vi "Player_Move.vi"(0 "State":T1={"Tick"=0, "Phase"=0, "PhaseTicks"=0, "Level"=1, "Room"=0, "X10"=0, "Y10"=0, "VY10"=0, "Mode"=0, "Facing"=0, "Run"=0, "Vert"=0, "StandY"=0, "EntryX10"=0, "EntryY10"=0, "EntryMode"=0, "Lives"=4, "Score"=0, "NextLife"=10000, "KeyR"=0, "KeyB"=0, "KeyY"=0, "Torch"=FALSE, "FloorPhase"=0, "Dead"=FALSE, "LevelStart"=FALSE, "Quit"=FALSE, "Sound"=0, "Seed"=12345, "DemoStep"=0, "Tiles"=[], "World"=[], "Enemies"=[], "Highscores"=[], "Name"=[0, 0, 0], "Cursor"=0}, 5 "Jump":bool, 11 "error in":errorcluster) -> (4 "State out":T1={"Tick"=0, "Phase"=0, "PhaseTicks"=0, "Level"=1, "Room"=0, "X10"=0, "Y10"=0, "VY10"=0, "Mode"=0, "Facing"=0, "Run"=0, "Vert"=0, "StandY"=0, "EntryX10"=0, "EntryY10"=0, "EntryMode"=0, "Lives"=4, "Score"=0, "NextLife"=10000, "KeyR"=0, "KeyB"=0, "KeyY"=0, "Torch"=FALSE, "FloorPhase"=0, "Dead"=FALSE, "LevelStart"=FALSE, "Quit"=FALSE, "Sound"=0, "Seed"=12345, "DemoStep"=0, "Tiles"=[], "World"=[], "Enemies"=[], "Highscores"=[], "Name"=[0, 0, 0], "Cursor"=0}, 15 "error out":errorcluster)   [LabVIEW 2020, in "GH_Engine.lvlib"]
doc: "Moves Claude by one tick: the step sideways (walking in Mode 0 and 2, conveyor push in Mode 0, stopped by a wall), then the mode: Move_Ground (0), Move_Ladder (1), Move_Air (2) or Move_Pole (3), all inline. Facing follows Run; StandY = last firm stand (for the fall height). Positions are tenths of a pixel."
uses:
  GH_Engine.lvlib
  Level/GH_Level.lvlib
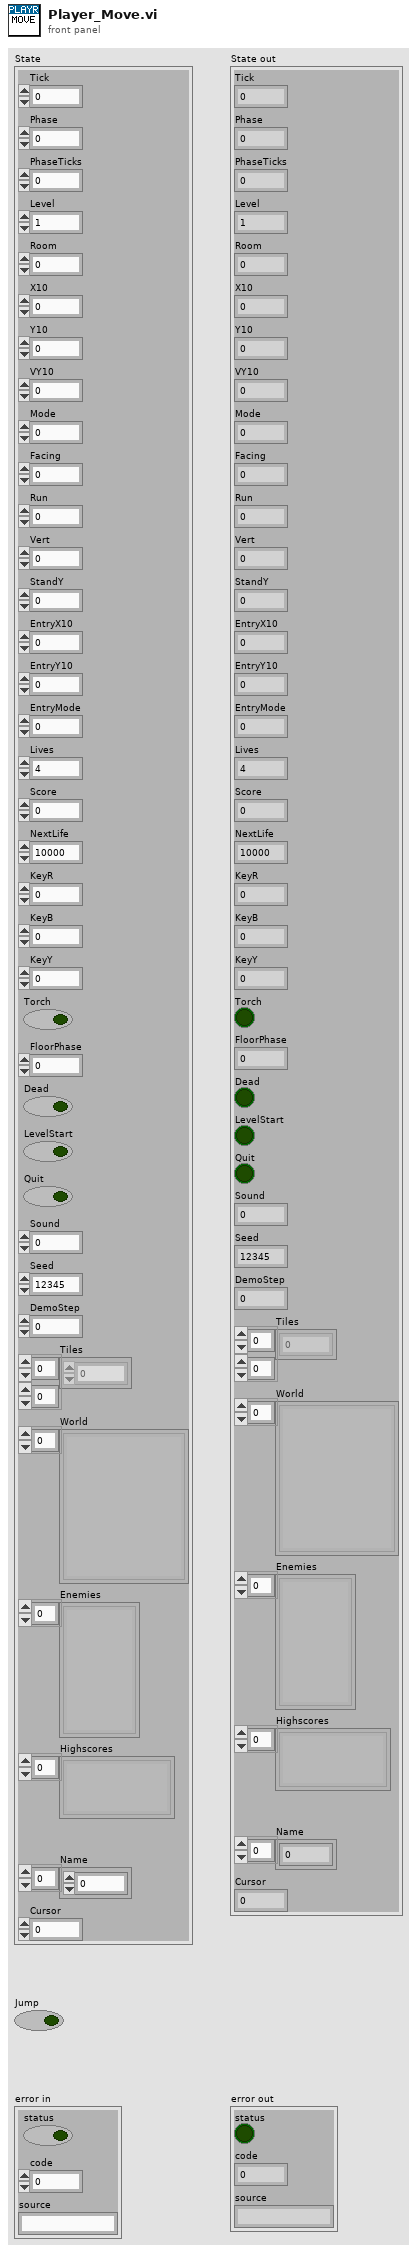
[diagram p1: front panel]
types:
  T1 = cluster{"Tick":u32, "Phase":i32, "PhaseTicks":i32, "Level":i32, "Room":i32, "X10":i32, "Y10":i32, "VY10":i32, "Mode":i32, "Facing":i32, "Run":i32, "Vert":i32, "StandY":i32, "EntryX10":i32, "EntryY10":i32, "EntryMode":i32, "Lives":i32, "Score":i32, "NextLife":i32, "KeyR":i32, "KeyB":i32, "KeyY":i32, "Torch":bool, "FloorPhase":i32, "Dead":bool, "LevelStart":bool, "Quit":bool, "Sound":i32, "Seed":u32, "DemoStep":i32, "Tiles":u8[][], "World":cluster{"ID":string, "Depth":i32, "Column":i32, "Tiles":u8[][]}[], "Enemies":cluster{"Kind":i32, "X10":i32, "Y10":i32, "Dir":i32, "Mode":i32}[], "Highscores":cluster{"Score":i32, "Name":string}[], "Name":i32[], "Cursor":i32}
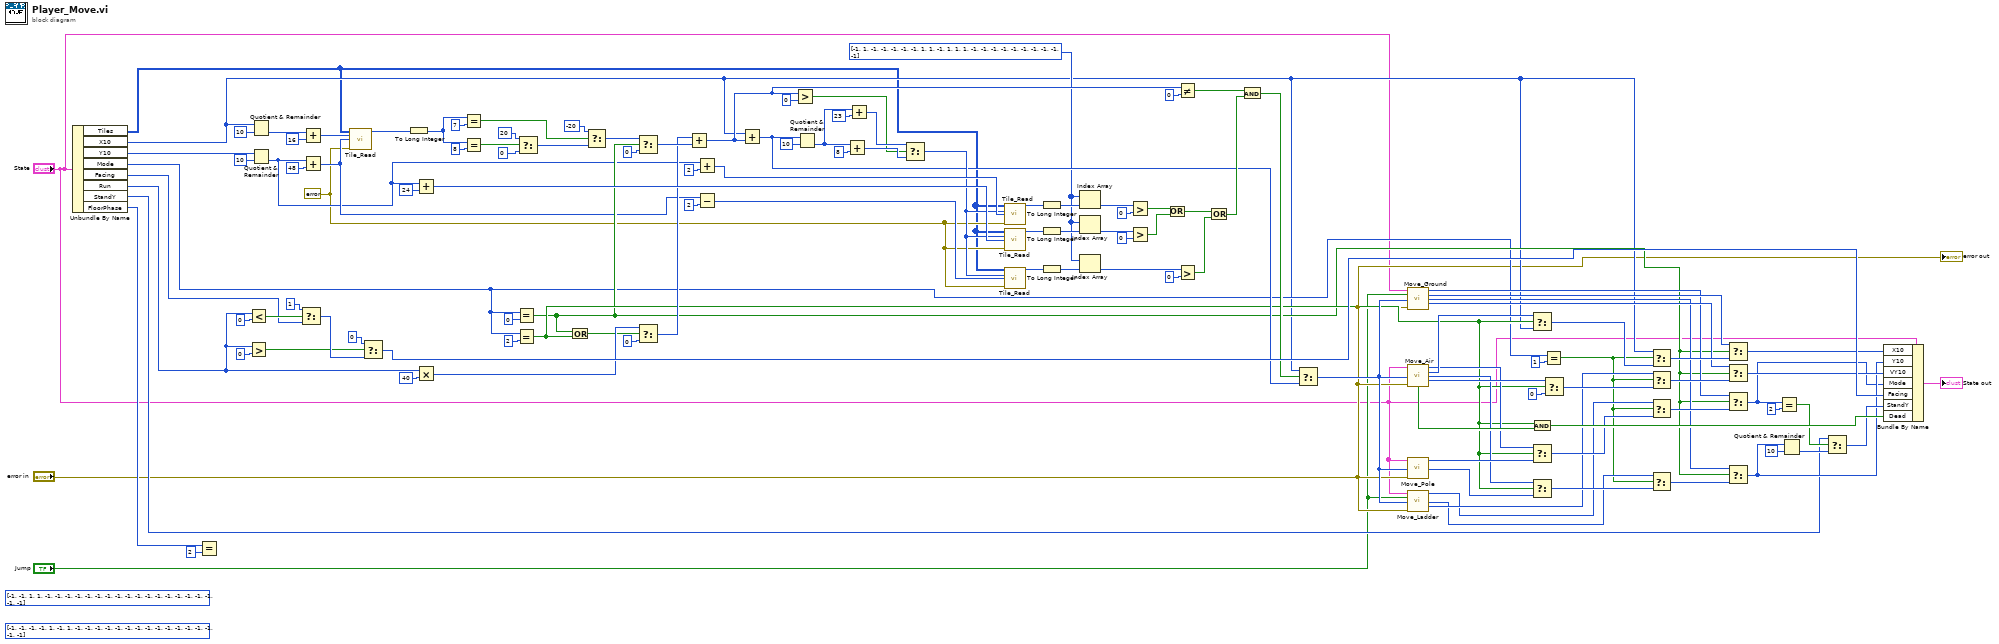
[diagram p0: block diagram]
diagram:
  w14 = errorcluster {"status"=FALSE, "code"=0, "source"=""} ("no error")
  (unwired) i32[] [-1, -1, -1, -1, 1, -1, 1, -1, -1, -1, -1, -1, -1, -1, -1, -1, -1, -1, -1, -1, -1, -1, -1] ("Ladder or rope")
  (unwired) i32[] [-1, -1, 1, 1, -1, -1, -1, -1, -1, -1, -1, -1, -1, -1, -1, -1, -1, -1, -1, -1, -1, -1, -1] ("Thin floor")
  w12 = i32[] [-1, 1, -1, -1, -1, -1, -1, 1, 1, -1, 1, 1, 1, -1, -1, -1, -1, -1, -1, -1, -1, -1, -1] ("Solid")
  n1 = Unbundle By Name("State") -> ("Tiles"=w4:u8[][], "X10"=w5:i32, "Y10"=w6:i32, "Mode"=w7:i32, "Facing"=w8:i32, "Run"=w9:i32, "StandY"=w10:i32, "FloorPhase"=w11:i32)
  n2 = Equal?(x=w11, y=2) -> ()  [unwired: 1 out]
  n3 = Less?(x=w9, y=0) -> (x < y?=w121:bool)
  n4 = Greater?(x=w9, y=0) -> (0:w118:bool)
  n5 = Quotient & Remainder(x=w5, y=10) -> (floor(x/y)=w16:i32)  [unwired: 1 out]
  n6 = Quotient & Remainder(x=w6, y=10) -> (floor(x/y)=w18:i32)  [unwired: 1 out]
  n7 = Select(t=1, s=w121, f=w8) -> (s? t:f=w123:i32)
  n8 = Add(x=w16, y=16) -> (x+y=w28:i32)
  n9 = Add(x=w18, y=48) -> (x+y=w20:i32)
  n10 = call "Tile_Read.vi"("Tiles"=w4, "X"=w28, "Y"=w20, "error in"=w14) -> ("Tile"=w29:u8)  [unwired: 10 in, 1 out]
  n11 = Select(t=0, s=w118, f=w123) -> (s? t:f=w124:i32)
  n12 = To Long Integer(number=w29) -> (32bit integer=w30:i32)
  n13 = Add(x=w18, y=24) -> (x+y=w66:i32)
  n14 = Multiply(x=w9, y=40) -> (x*y=w42:i32)
  n15 = Equal?(x=w30, y=7) -> (x = y?=w32:bool)
  n16 = Equal?(x=w30, y=8) -> (x = y?=w35:bool)
  n17 = Equal?(x=w7, y=0) -> (x = y?=w22:bool)
  n18 = Equal?(x=w7, y=2) -> (x = y?=w26:bool)
  n19 = Select(t=20, s=w35, f=0) -> (s? t:f=w38:i32)
  n20 = Or(x=w22, y=w26) -> (x .or. y?=w40:bool)
  n21 = Select(t=-20, s=w32, f=w38) -> (s? t:f=w39:i32)
  n22 = Select(t=w39, s=w22, f=0) -> (s? t:f=w46:i32)
  n23 = Select(t=w42, s=w40, f=0) -> (s? t:f=w44:i32)
  n24 = Add(x=w44, y=w46) -> (x+y=w47:i32)
  n25 = Add(x=w18, y=2) -> (x+y=w59:i32)
  n26 = Subtract(x=w20, y=2) -> (x-y=w73:i32)
  n27 = Add(x=w5, y=w47) -> (x+y=w48:i32)
  n28 = Greater?(x=w47, y=0) -> (0:w52:bool)
  n29 = Quotient & Remainder(x=w48, y=10) -> (floor(x/y)=w50:i32)  [unwired: 1 out]
  n30 = Add(x=w50, y=8) -> (x+y=w56:i32)
  n31 = Add(x=w50, y=23) -> (x+y=w54:i32)
  n32 = Select(t=w54, s=w52, f=w56) -> (s? t:f=w57:i32)
  n33 = call "Tile_Read.vi"("Tiles"=w4, "X"=w57, "Y"=w59, "error in"=w14) -> ("Tile"=w60:u8)  [unwired: 10 in, 1 out]
  n34 = call "Tile_Read.vi"("Tiles"=w4, "X"=w57, "Y"=w66, "error in"=w14) -> ("Tile"=w67:u8)  [unwired: 10 in, 1 out]
  n35 = call "Tile_Read.vi"("Tiles"=w4, "X"=w57, "Y"=w73, "error in"=w14) -> ("Tile"=w74:u8)  [unwired: 10 in, 1 out]
  n36 = To Long Integer(number=w60) -> (32bit integer=w61:i32)
  n37 = To Long Integer(number=w67) -> (32bit integer=w68:i32)
  n38 = To Long Integer(number=w74) -> (32bit integer=w75:i32)
  n39 = Index Array(array=w12, index=w61) -> (element=w62:i32)
  n40 = Index Array(array=w12, index=w68) -> (element=w69:i32)
  n41 = Index Array(array=w12, index=w75) -> (element=w76:i32)
  n42 = Greater?(x=w62, y=0) -> (0:w64:bool)
  n43 = Greater?(x=w69, y=0) -> (0:w71:bool)
  n44 = Or(x=w64, y=w71) -> (x .or. y?=w79:bool)
  n45 = Not Equal?(x=w47, y=0) -> (x != y?=w82:bool)
  n46 = Greater?(x=w76, y=0) -> (0:w78:bool)
  n47 = Or(x=w79, y=w78) -> (x .or. y?=w80:bool)
  n48 = And(x=w82, y=w80) -> (x .and. y?=w83:bool)
  n49 = Select(t=w5, s=w83, f=w48) -> (s? t:f=w84:i32)
  n50 = call "Move_Ground.vi"("State"="State", "Jump"="Jump", "XA10"=w84, "error in"="error in") -> ("Mode"=w85:i32, "X10"=w86:i32, "Y10"=w87:i32, "VY10"=w88:i32)  [unwired: 7 in, 1 out]
  n51 = call "Move_Air.vi"("State"="State", "XA10"=w84, "error in"="error in") -> ("Mode"=w89:i32, "X10"=w90:i32, "Y10"=w91:i32, "VY10"=w92:i32, "Dead"=w93:bool)  [unwired: 7 in, 1 out]
  n52 = call "Move_Pole.vi"("State"="State", "XA10"=w84, "error in"="error in") -> ("Mode"=w97:i32, "Y10"=w98:i32)  [unwired: 10 in, 1 out]
  n53 = call "Move_Ladder.vi"("State"="State", "Jump"="Jump", "XA10"=w84, "error in"="error in") -> ("Mode"=w94:i32, "Y10"=w95:i32, "VY10"=w96:i32)  [unwired: 8 in, 1 out]
  n54 = Select(t=w90, s=w26, f=w5) -> (s? t:f=w102:i32)
  n55 = Select(t=w89, s=w26, f=w97) -> (s? t:f=w99:i32)
  n56 = Select(t=w91, s=w26, f=w98) -> (s? t:f=w105:i32)
  n57 = And(x=w26, y=w93) -> (x .and. y?=w125:bool)
  n58 = Equal?(x=w7, y=1) -> (x = y?=w24:bool)
  n59 = Select(t=w92, s=w26, f=0) -> (s? t:f=w109:i32)
  n60 = Select(t=w5, s=w24, f=w102) -> (s? t:f=w103:i32)
  n61 = Select(t=w96, s=w24, f=w109) -> (s? t:f=w110:i32)
  n62 = Select(t=w94, s=w24, f=w99) -> (s? t:f=w100:i32)
  n63 = Select(t=w95, s=w24, f=w105) -> (s? t:f=w106:i32)
  n64 = Select(t=w86, s=w22, f=w103) -> (s? t:f=w104:i32)
  n65 = Select(t=w88, s=w22, f=w110) -> (s? t:f=w111:i32)
  n66 = Select(t=w85, s=w22, f=w100) -> (s? t:f=w101:i32)
  n67 = Select(t=w87, s=w22, f=w106) -> (s? t:f=w107:i32)
  n68 = Equal?(x=w101, y=2) -> (x = y?=w113:bool)
  n69 = Quotient & Remainder(x=w107, y=10) -> (floor(x/y)=w115:i32)  [unwired: 1 out]
  n70 = Select(t=w10, s=w113, f=w115) -> (s? t:f=w116:i32)
  n71 = Bundle By Name(cluster="State", "X10"=w104, "Y10"=w107, "VY10"=w111, "Mode"=w101, "Facing"=w124, "StandY"=w116, "Dead"=w125) -> (→"State out":T1)
  "error out" <- "error in"
